vi "Load Config.vi"(8 "error in (no error)":errorcluster, 11 "DAQmxThermocoupleChannel in":refnum<class "TCChannel.lvclass">) -> (0 "error out":errorcluster, 3 "DAQmxThermocoupleChannel out":refnum<class "TCChannel.lvclass">)   [LabVIEW 2020, in "VolatusDAQConfig.lvlib" / "TCChannel.lvclass"]
uses:
  TCChannel.lvclass
  C:/dev/lv20CE/relink/lv-volatus/VolatusConfig/VolatusConfigElement/VolatusConfigElement.lvclass
  Temperature Units.ctl
  TC Type.ctl
  VolatusConfig/VolatusConfigElement/VolatusConfigElement.lvclass/VolatusConfigElement.ctl
  TCChannel.lvclass/TCChannel.ctl
  VolatusConfig/VolatusConfigElement/Element.vi
  VolatusConfig/VolatusConfigElement/VolatusConfigElement.lvclass
  lv-cdm/CDM-Config/Config Element/Config Element.lvclass
  VolatusDAQConfig.lvlib
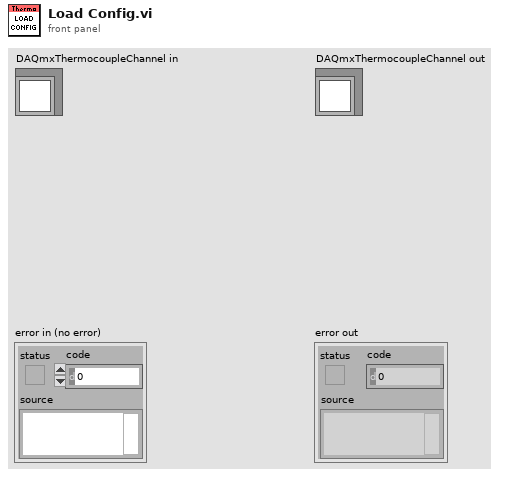
[diagram p1: front panel]
types:
  T1 = typedef "VolatusDAQConfig.lvlib/TC Type.ctl" = enum16{"J", "K", "N", "R", "S", "T", "B", "E"}
  T2 = typedef "VolatusDAQConfig.lvlib/Temperature Units.ctl" = enum16{"C", "F", "K", "R"}
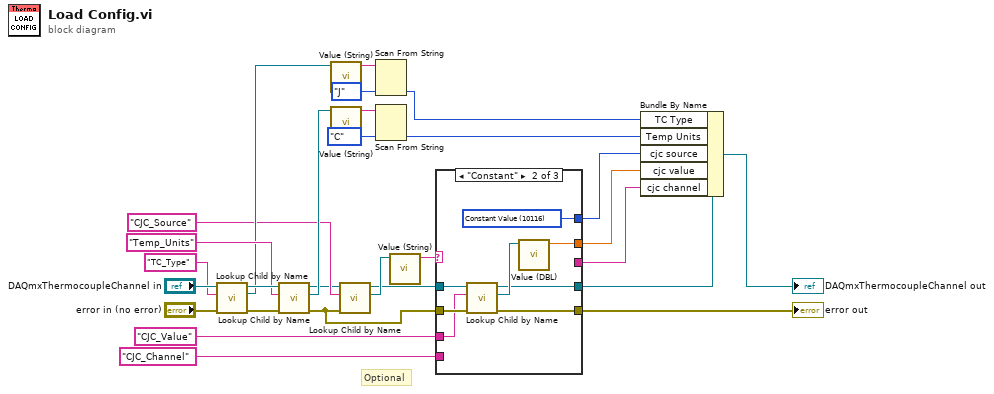
[diagram p0: block diagram]
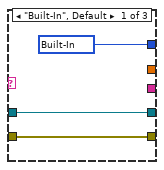
[diagram p2: hidden frame]
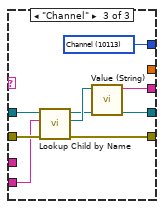
[diagram p3: hidden frame]
diagram:
  # "Optional"
  n1 = call "Lookup Child by Name.vi"("error in (no error)"="error in (no error)", "Child Name"="TC_Type", "VolatusConfigElement in"="DAQmxThermocoupleChannel in") -> ("error out"=w27:errorcluster, "Child"=w22:refnum<class "Config Element.lvclass">, "VolatusConfigElement out"=w24:refnum<class "TCChannel.lvclass">)  [unwired: 5 in, 1 out]
  n2 = call "Lookup Child by Name.vi"("error in (no error)"=w27, "Child Name"="Temp_Units", "VolatusConfigElement in"=w24) -> ("error out"=w1:errorcluster, "Child"=w21:refnum<class "Config Element.lvclass">, "VolatusConfigElement out"=w13:refnum<class "TCChannel.lvclass">)  [unwired: 5 in, 1 out]
  n3 = call "Value (String).vi"("Config Element in"=w22) -> ("String Value"=w18:string)  [unwired: 9 in, 1 out]
  n4 = call "Value (String).vi"("Config Element in"=w21) -> ("String Value"=w20:string)  [unwired: 9 in, 1 out]
  n5 = call "Lookup Child by Name.vi"("error in (no error)"=w1, "Child Name"="CJC_Source", "VolatusConfigElement in"=w13) -> ("Child"=w12:refnum<class "Config Element.lvclass">, "VolatusConfigElement out"=w10:refnum<class "TCChannel.lvclass">)  [unwired: 5 in, 2 out]
  n6 = Scan From String(input string=w18, default 1=TC_Type."J" ("TC Type")) -> (output 1=w15:T1)  [unwired: 3 in, 3 out]
  n7 = Scan From String(input string=w20, default 1=Temperature_Units."C" ("Temp Units")) -> (output 1=w16:T2)  [unwired: 3 in, 3 out]
  n8 = call "Value (String).vi"("Config Element in"=w12) -> ("String Value"=w11:string)  [unwired: 9 in, 1 out]
  n9 = case shown="\"Constant\"" w11 {
    tunnel: w10 -> [w30 w39 w47]
    tunnel: w1 -> [w29 w38 w46]
    tunnel: "CJC_Value" ("Child Name") -> [_ w37 _]
    tunnel: [w29 w35 w44] -> w8
    tunnel: [w30 w34 w43] -> w6
    tunnel: [w31 w33 w42] -> w7
    tunnel: [_ w32 _] -> w4
    tunnel: "CJC_Channel" ("Child Name") -> [_ _ w41]
    tunnel: [_ _ w40] -> w2
    frame "Built-In", Default {
      w31 = 10200 items=["Built-In"=10200, "Constant Value"=10116, "Channel"=10113] ("cjc source")
    }
    frame "Constant" {
      w33 = 10116 items=["Built-In"=10200, "Constant Value"=10116, "Channel"=10113] ("cjc source")
      n10 = call "Lookup Child by Name.vi"("error in (no error)"=w38, "Child Name"=w37, "VolatusConfigElement in"=w39) -> ("error out"=w35:errorcluster, "Child"=w36:refnum<class "Config Element.lvclass">, "VolatusConfigElement out"=w34:refnum<class "TCChannel.lvclass">)  [unwired: 5 in, 1 out]
      n11 = call "Value (DBL).vi"("Config Element in"=w36) -> ("DBL Value"=w32:dbl)  [unwired: 9 in, 1 out]
    }
    frame "Channel" {
      w42 = 10113 items=["Built-In"=10200, "Constant Value"=10116, "Channel"=10113] ("cjc source")
      n12 = call "Lookup Child by Name.vi"("error in (no error)"=w46, "Child Name"=w41, "VolatusConfigElement in"=w47) -> ("error out"=w44:errorcluster, "Child"=w45:refnum<class "Config Element.lvclass">, "VolatusConfigElement out"=w43:refnum<class "TCChannel.lvclass">)  [unwired: 5 in, 1 out]
      n13 = call "Value (String).vi"("Config Element in"=w45) -> ("String Value"=w40:string)  [unwired: 9 in, 1 out]
    }
  }
  "error out" <- w8
  n14 = Bundle By Name(cluster=w6, "TC Type"=w15, "Temp Units"=w16, "cjc source"=w7, "cjc value"=w4, "cjc channel"=w2) -> (→"DAQmxThermocoupleChannel out":refnum<class "TCChannel.lvclass">)
